vi "name_path.vi"(5 "Suffix":string, 6 "error in name_subvi":errorcluster, 7 "Speed RPM":dbl, 8 "Power W":dbl, 9 "Resistor":dbl, 10 "Arms":dbl, 11 "Base Folder":path) -> (0 "error out name_subvi":errorcluster, 3 "File Path":path)   [LabVIEW 2025]
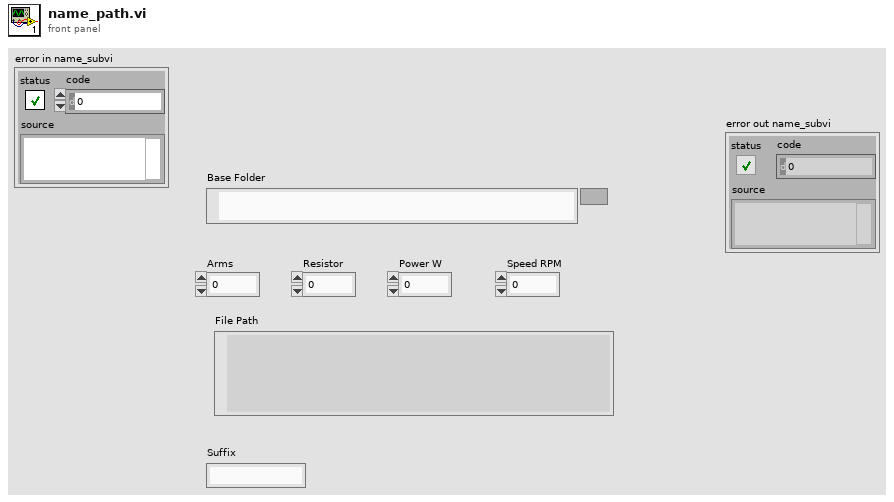
[diagram p1: front panel]
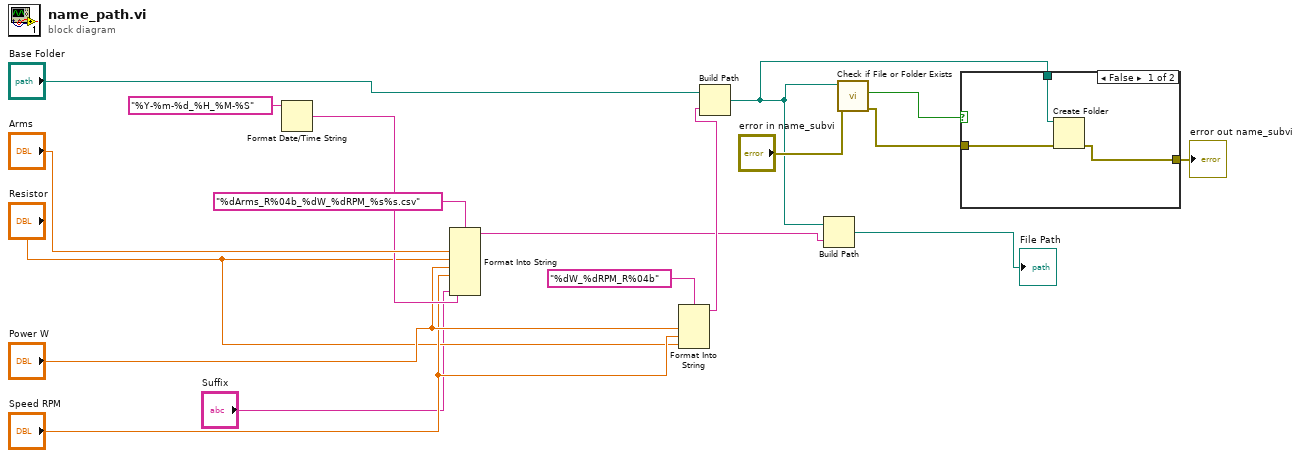
[diagram p0: block diagram]
diagram:
  n1 = Format Date/Time String(time format string (%c)="%Y-%m-%d_%H_%M-%S") -> (date/time string=w15:string)  [unwired: 2 in]
  n2 = Format Into String(format string="%dArms_R%04b_%dW_%dRPM_%s%s.csv", "Arms", "Resistor", "Power W", "Speed RPM", w15, "Suffix") -> (resulting string=w3:string)  [unwired: 2 in, 1 out]
  n3 = Format Into String(format string="%dW_%dRPM_R%04b", "Power W", "Speed RPM", "Resistor") -> (resulting string=w9:string)  [unwired: 2 in, 1 out]
  n4 = Build Path(base path="Base Folder", name or relative path=w9) -> (appended path=w4:path)
  n5 = Build Path(base path=w4, name or relative path=w3) -> (appended path=→"File Path":path)
  n6 = call <vilib>:"Check if File or Folder Exists.vi"("error in (no error)"="error in name_subvi", "path"=w4) -> ("error out"=w6:errorcluster, "file or folder exists?"=w7:bool)  [unwired: 7 in, 1 out]
  n7 = case shown="False" w7 {
    tunnel: w4 -> [w21 _]
    tunnel: w6 -> [w20 w22]
    tunnel: [w19 w22] -> w5
    frame False {
      n8 = Create Folder(path (use dialog)=w21, error in=w20) -> (error out=w19:errorcluster)  [unwired: 1 in, 2 out]
    }
    frame True {
    }
  }
  "error out name_subvi" <- w5
